vi "Substitute Class.vi"(8 "error in (no error)":errorcluster, 10 "New Class":path=path "C:/temp/Test2/Test2.lvclass", 11 "Class to Replace":path=path "C:/temp/Test1.lvclass") -> (0 "error out":errorcluster)   [LabVIEW 2020, in "Mock Class Updater.lvclass"]
uses:
  Mock Class Updater.lvclass
  Mock Class Updater.lvclass/Mock Class Updater.ctl
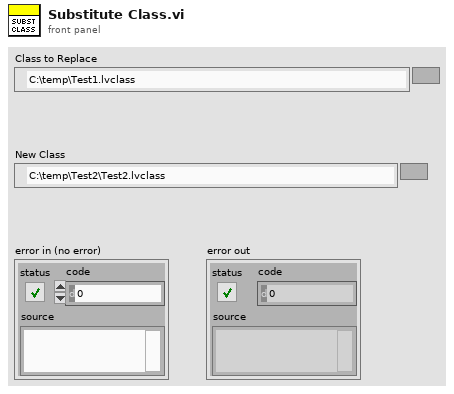
[diagram p1: front panel]
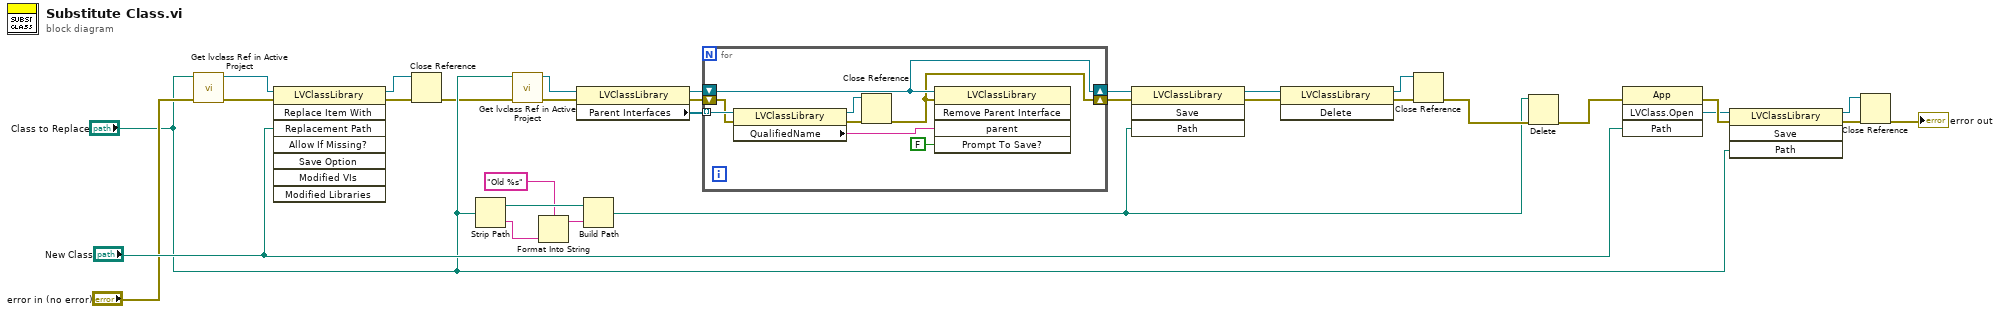
[diagram p0: block diagram]
diagram:
  n1 = call "Get lvclass Ref in Active Project.vi"("error in (no error)"="error in (no error)", "File"="Class to Replace") -> ("error out"=w24:errorcluster, "LVClassLibrary out"=w25:refnum<vi>)  [unwired: 8 in]
  n2 = invoke class="LVClassLibrary" method="Replace Item With"(reference=w25, error in=w24, "Replacement Path"="New Class") -> (reference out=w19:refnum<vi>, error out=w22:errorcluster)  [unwired: 5 in, 6 out]
  n3 = Close Reference(reference=w19, error in (no error)=w22) -> (error out=w15:errorcluster)
  n4 = Strip Path(path="Class to Replace") -> (stripped path=w20:path, name=w11:string)
  n5 = call "Get lvclass Ref in Active Project.vi"("error in (no error)"=w15, "File"="Class to Replace") -> ("error out"=w14:errorcluster, "LVClassLibrary out"=w5:refnum<vi>)  [unwired: 8 in]
  n6 = Format Into String(format string="Old %s", w11) -> (resulting string=w10:string)  [unwired: 2 in, 1 out]
  n7 = property class="LVClassLibrary"(reference=w5, error in=w14) -> (reference out=w3:refnum<vi>, error out=w6:errorcluster, "Parent Interfaces"=w1:refnum<vi>[])
  n8 = Build Path(base path=w20, name or relative path=w10) -> (appended path=w7:path)
  n9 = for {
    tunnel: w1 -> [w38] mode=indexing
    shift-right: [w32] -> w4
    shift-left: w6 -> [w36]
    shift-right: [w33] -> w2
    shift-left: w3 -> [w33]
    n10 = property class="LVClassLibrary"(reference=w38, error in=w36) -> (reference out=w34:refnum<vi>, error out=w35:errorcluster, "QualifiedName"=w37:string)
    n11 = Close Reference(reference=w34, error in (no error)=w35) -> (error out=w32:errorcluster)
    n12 = invoke class="LVClassLibrary" method="Remove Parent Interface"(reference=w33, error in=w32, "parent"=w37, "Prompt To Save?"=FALSE) -> ()  [unwired: 1 in, 5 out]
  }
  n13 = invoke class="LVClassLibrary" method="Save"(reference=w2, error in=w4, "Path"=w7) -> (reference out=w17:refnum<vi>, error out=w21:errorcluster)  [unwired: 1 in, 2 out]
  n14 = invoke class="LVClassLibrary" method="Delete"(reference=w17, error in=w21) -> (reference out=w13:refnum<vi>, error out=w18:errorcluster)  [unwired: 1 in, 1 out]
  n15 = Close Reference(reference=w13, error in (no error)=w18) -> (error out=w9:errorcluster)
  n16 = Delete(path (use dialog)=w7, error in=w9) -> (error out=w8:errorcluster)  [unwired: 3 in, 2 out]
  n17 = invoke class="App" method="LVClass.Open"(error in=w8, "Path"="New Class") -> (error out=w27:errorcluster, "LVClass.Open"=w26:refnum<vi>)  [unwired: 2 in, 2 out]
  n18 = invoke class="LVClassLibrary" method="Save"(reference=w26, error in=w27, "Path"="Class to Replace") -> (reference out=w30:refnum<vi>, error out=w28:errorcluster)  [unwired: 1 in, 2 out]
  n19 = Close Reference(reference=w30, error in (no error)=w28) -> (error out=→"error out":errorcluster)
